vi "Shutdown.vi"(8 "error in (no error)":errorcluster, 11 "VolatusAPI in":refnum<class "VolatusAPI.lvclass">) -> (0 "error out":errorcluster, 3 "VolatusAPI out":refnum<class "VolatusAPI.lvclass">)   [LabVIEW 2020, in "Volatus.lvlib" / "VolatusAPI.lvclass"]
uses:
  VolatusAPI.lvclass
  Volatus Core Identity/Volatus Core Identity.lvclass
  C:/dev/lv20CE/relink/lv-volatus/Volatus/Identity/Identity.lvclass
  VolatusAPI.lvclass/VolatusAPI.ctl
  Volatus.lvlib
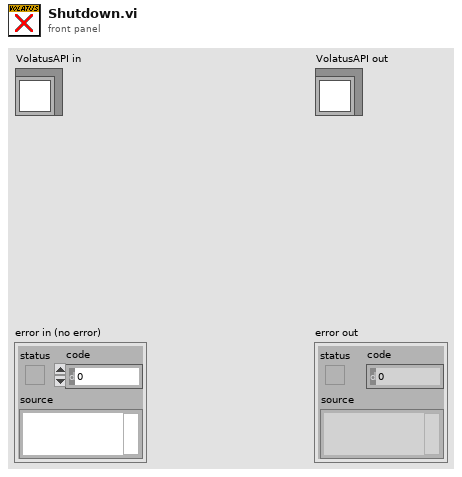
[diagram p1: front panel]
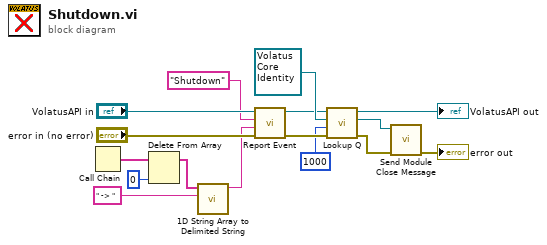
[diagram p0: block diagram]
diagram:
  n1 = Call Chain() -> (call chain=w6:string[])
  n2 = Delete From Array(array=w6, index=0) -> (array with subset deleted=w3:string[])  [unwired: 1 in, 1 out]
  n3 = call <vilib>:"1D String Array to Delimited String.vi"("delimiter"=" -> ", "string array"=w3) -> ("delimited string"=w4:string)  [unwired: 9 in]
  n4 = call "Report Event.vi"("error in (no error)"="error in (no error)", "Message"=w4, "Context"="Shutdown", "VolatusAPI in"="VolatusAPI in") -> ("error out"=w16:errorcluster, "VolatusAPI out"=w8:refnum<class "VolatusAPI.lvclass">)  [unwired: 6 in]
  n5 = call "Lookup Q.vi"("error in (no error)"=w16, "Timeout ms (0)"=1000, "Identity"=refnum<class "Volatus Core Identity.lvclass"> refnum ("Volatus:Volatus Core Identity.lvclass"), "VolatusAPI in"=w8) -> ("error out"=w12:errorcluster, "MessageQ"=w13:refnum<class "MessageQ.lvclass">, "VolatusAPI out"=→"VolatusAPI out":refnum<class "VolatusAPI.lvclass">)  [unwired: 5 in]
  n6 = call "Send Module Close Message.vi"("error in (no error)"=w12, "MessageQ"=w13) -> ("error out"=→"error out":errorcluster)  [unwired: 9 in]
